vi "REG 1COM-MODBUS.vi"(3 "N° port COM":u8) -> (1 "cluster de sortie":cluster{string[][]})   [LabVIEW 2022 SP3]
uses:
  Variables globales/Variables glob EUROTHERM.vi
  Variables globales/Variable glob generale.vi
panel:
  out "data reg":string[](array[string])
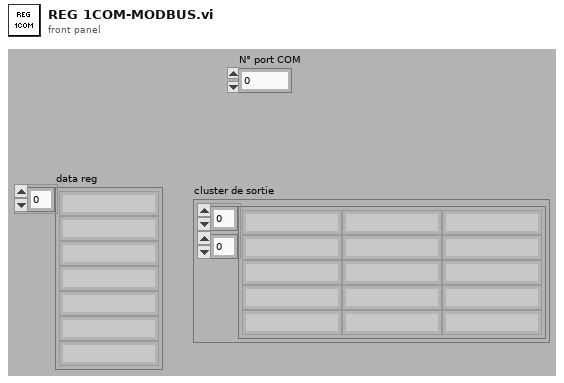
[diagram p1: front panel]
types:
  T1 = cluster{"Baud Rate (9600)":u32, "Parity (0: None)":u16, "Break Length (0)":u16}
  T2 = typedef "Semaphore RefNum" = refnum<k1>
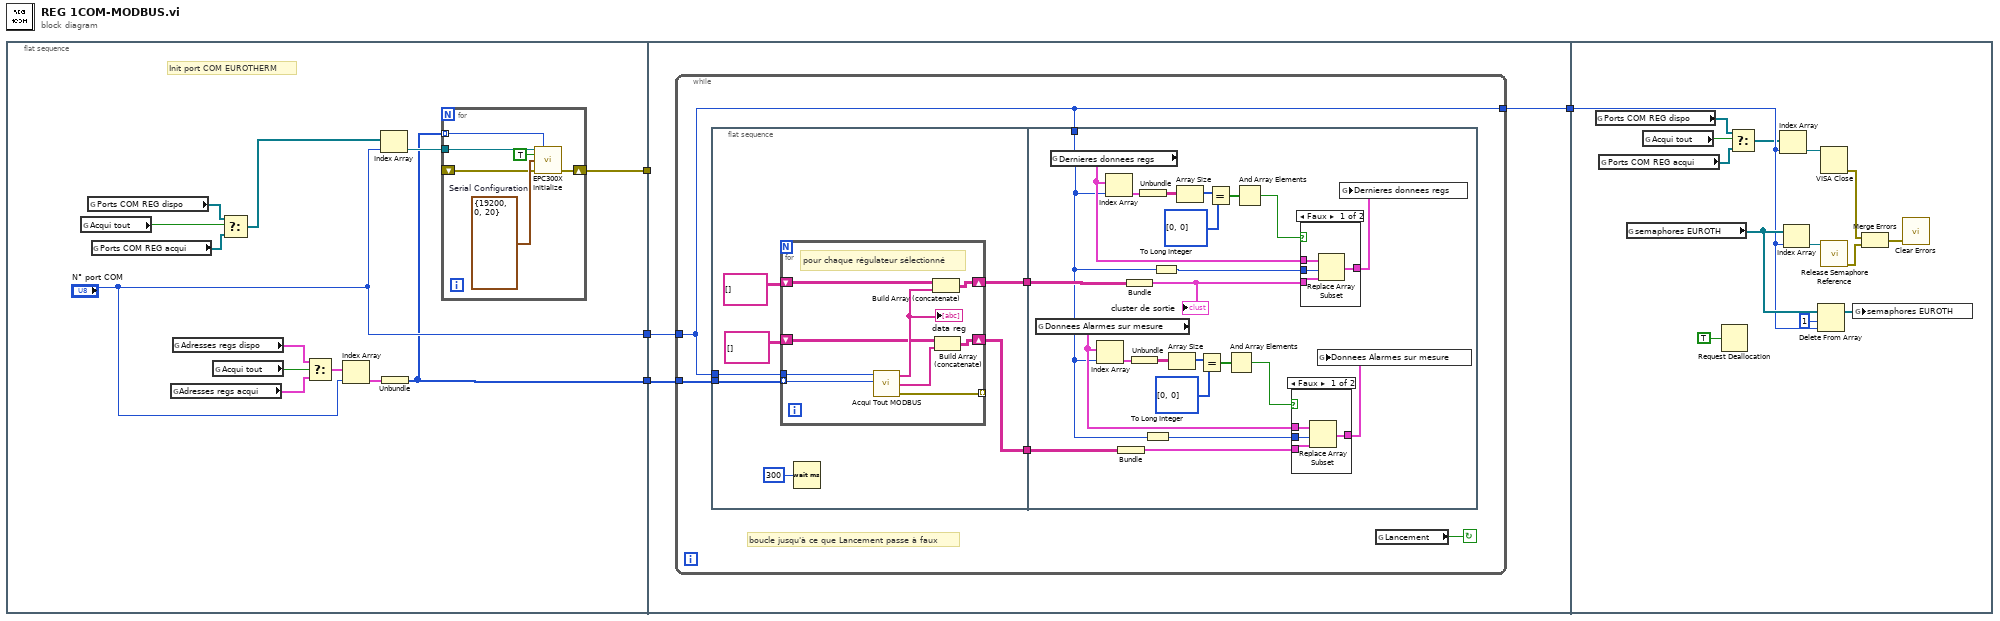
[diagram p0: block diagram]
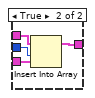
[diagram p2: hidden frame]
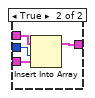
[diagram p3: hidden frame]
diagram:
  n1 = flat-sequence {
    tunnel: ["N° port COM"] -> w4
    tunnel: [w6] -> w3
    tunnel: [w5] -> w1
    tunnel: w4 -> [w26]
    tunnel: w3 -> [w25]
    tunnel: [w24] -> w2
    tunnel: w1 -> [_]
    tunnel: w2 -> [w92]
    frame #0 {
      # "Init port COM EUROTHERM"
      n2 = global read "Variable glob generale.vi" "Acqui tout"() -> (w8:bool)
      n3 = global read "Variables glob EUROTHERM.vi" "Ports COM REG dispo"() -> (w11:refnum<visa-resource-name>[])
      n4 = global read "Variables glob EUROTHERM.vi" "Ports COM REG acqui"() -> (w10:refnum<visa-resource-name>[])
      n5 = global read "Variables glob EUROTHERM.vi" "Adresses regs acqui"() -> (w13:cluster{"Adresses acqui 1COM reg":u16[]}[])
      n6 = global read "Variables glob EUROTHERM.vi" "Adresses regs dispo"() -> (w14:cluster{"Adresses 1COM reg":u16[]}[])
      n7 = global read "Variable glob generale.vi" "Acqui tout"() -> (w15:bool)
      n8 = Select(t=w11, s=w8, f=w10) -> (s? t:f=w9:refnum<visa-resource-name>[])
      n9 = Select(t=w14, s=w15, f=w13) -> (s? t:f=w12:cluster{"Adresses acqui 1COM reg":u16[]}[])
      n10 = Index Array(array=w12, index="N° port COM") -> (element=w17:cluster{"Adresses acqui 1COM reg":u16[]})
      n11 = Index Array(array=w9, index="N° port COM") -> (element=w7:refnum<visa-resource-name>)
      n12 = Unbundle(w17) -> ("Adresses acqui 1COM reg"=w6:u16[])
      n13 = for {
        tunnel: w7 -> [w23]
        tunnel: w6 -> [w20] mode=indexing
        shift-right: [w19] -> w5
        shift-left: _ -> [w18]
        w22 = T1 {"Baud Rate (9600)"=19200, "Parity (0: None)"=0, "Break Length (0)"=20}  # Serial Configuration
        n14 = call "EPC300X Initialize.vi"("VISA resource name"=w23, "Unit Address (1)"=w20, "ID Query? (T: Yes)"=TRUE, "Serial Configuration"=w22, "error in (no error)"=w18) -> ("error out"=w19:errorcluster)  [unwired: 9 in, 1 out]
      }
    }
    frame #1 {
      n15 = while {
        tunnel: w26 -> [w28]
        tunnel: w25 -> [w30]
        tunnel: [w28] -> w24
        stop <- w31 continue-if-true
        # "boucle jusqu'à ce que Lancement passe à faux"
        n16 = flat-sequence {
          tunnel: w30 -> [w36]
          tunnel: w28 -> [w35]
          tunnel: [w38] -> w29
          tunnel: [w32] -> w27
          tunnel: w29 -> [w60]
          tunnel: w28 -> [w48]
          tunnel: w27 -> [w49]
          frame #0 {
            n17 = for {
              tunnel: w36 -> [w46] mode=indexing
              tunnel: w35 -> [w47]
              shift-right: [w44] -> w38
              shift-left: string[][] [] -> [w45]
              tunnel: [w42] -> _ mode=indexing
              shift-right: [w41] -> w32
              shift-left: string[][] [] -> [w40]
              # "pour chaque régulateur sélectionné"
              n18 = call "Acqui Tout MODBUS.vi"("Adresse régulateur"=w46, "Port COM"=w47) -> ("error out"=w42:errorcluster, "Al sur mesure"=w39:string[], "data reg"=w43:string[])  [unwired: 2 in]
              "data reg" <- w43
              n19 = Build Array (concatenate)(w45, w43) -> (w44:string[][])
              n20 = Build Array (concatenate)(w40, w39) -> (w41:string[][])
            }
            n21 = Wait (ms)(milliseconds to wait=u32 300 ("n millisecondes")) -> ()  [unwired: 1 out]
          }
          frame #1 {
            n22 = global read "Variables glob EUROTHERM.vi" "Donnees Alarmes sur mesure"() -> (w57:cluster{"AL sur mes 1COM":string[][]}[])
            n23 = global read "Variables glob EUROTHERM.vi" "Dernieres donnees regs"() -> (w63:cluster{"Dernieres donnees 1COM":string[][]}[])
            n24 = Index Array(array=w57, index=w48) -> (element=w59:cluster{"AL sur mes 1COM":string[][]})
            n25 = Index Array(array=w63, index=w48) -> (element=w61:cluster{"Dernieres donnees 1COM":string[][]})
            n26 = Bundle(w49) -> (w56:cluster{string[][]})  [unwired: 1 in]
            n27 = Bundle(w60) -> (w64:cluster{string[][]})  [unwired: 1 in]
            "cluster de sortie" <- w64
            n28 = Unbundle(w59) -> ("AL sur mes 1COM"=w55:string[][])
            n29 = Unbundle(w61) -> ("Dernieres donnees 1COM"=w65:string[][])
            n30 = To Long Integer(number=w48) -> (32bit integer=w50:i32)
            n31 = To Long Integer(number=w48) -> (32bit integer=w70:i32)
            n32 = Array Size(array=w55) -> (size(s)=w54:i32[])
            n33 = Array Size(array=w65) -> (size(s)=w66:i32[])
            n34 = Equal?(x=w54, y=i32[] [0, 0]) -> (x = y?=w53:bool[])
            n35 = Equal?(x=w66, y=i32[] [0, 0]) -> (x = y?=w67:bool[])
            n36 = And Array Elements(Boolean array=w53) -> (logical AND=w51:bool)
            n37 = And Array Elements(Boolean array=w67) -> (logical AND=w69:bool)
            n38 = case shown="Faux" w51 {
              tunnel: w56 -> [w74 w78]
              tunnel: [w73 w75] -> w58
              tunnel: w57 -> [w72 w77]
              tunnel: w50 -> [w71 w76]
              frame False {
                n39 = Replace Array Subset(array=w72, new element=w74, index=w71) -> (w73:cluster{"AL sur mes 1COM":string[][]}[])
              }
              frame True {
                n40 = Insert Into Array(array=w77, index=w76, new element=w78) -> (w75:cluster{"AL sur mes 1COM":string[][]}[])
              }
            }
            n41 = case shown="Faux" w69 {
              tunnel: w64 -> [w82 w86]
              tunnel: [w81 w83] -> w62
              tunnel: w63 -> [w80 w85]
              tunnel: w70 -> [w79 w84]
              frame False {
                n42 = Replace Array Subset(array=w80, new element=w82, index=w79) -> (w81:cluster{"Dernieres donnees 1COM":string[][]}[])
              }
              frame True {
                n43 = Insert Into Array(array=w85, index=w84, new element=w86) -> (w83:cluster{"Dernieres donnees 1COM":string[][]}[])
              }
            }
            n44 = global write "Variables glob EUROTHERM.vi" "Donnees Alarmes sur mesure"(w58) -> ()
            n45 = global write "Variables glob EUROTHERM.vi" "Dernieres donnees regs"(w62) -> ()
          }
        }
        n46 = global read "Variable glob generale.vi" "Lancement"() -> (w31:bool)
      }
    }
    frame #2 {
      n47 = global read "Variables glob EUROTHERM.vi" "Ports COM REG dispo"() -> (w89:refnum<visa-resource-name>[])
      n48 = global read "Variables glob EUROTHERM.vi" "Ports COM REG acqui"() -> (w90:refnum<visa-resource-name>[])
      n49 = global read "Variables glob EUROTHERM.vi" "semaphores EUROTH"() -> (w98:T2[])
      n50 = global read "Variable glob generale.vi" "Acqui tout"() -> (w88:bool)
      n51 = Request Deallocation(TRUE ("flag")) -> ()
      n52 = Select(t=w89, s=w88, f=w90) -> (s? t:f=w87:refnum<visa-resource-name>[])
      n53 = Index Array(array=w87, index=w92) -> (element=w96:refnum<visa-resource-name>)
      n54 = Index Array(array=w98, index=w92) -> (element=w97:T2)
      n55 = Delete From Array(array=w98, length=1 ("longueur"), index=w92) -> (array with subset deleted=w99:T2[])  [unwired: 1 out]
      n56 = VISA Close(VISA resource name=w96) -> (error out=w94:errorcluster)  [unwired: 1 in]
      n57 = call <vilib>:"Release Semaphore Reference.vi"("semaphore"=w97) -> ("error out"=w95:errorcluster)  [unwired: 9 in, 1 out]
      n58 = global write "Variables glob EUROTHERM.vi" "semaphores EUROTH"(w99) -> ()
      n59 = Merge Errors(w94, w95) -> (w91:errorcluster)
      n60 = call <vilib>:"Clear Errors.vi"("error in (no error)"=w91) -> ()  [unwired: 5 in, 2 out]
    }
  }
